vi "CANsub_Phy_Body.vi"(8 "error in (no error)":errorcluster, 11 "Bit_Timing":T1={"brp"=2, "seg1"=63, "seg2"=16, "sjw"=16, "data brp"=2, "data seg1"=15, "data seg2"=4, "data sjw"=4}) -> (0 "error out":errorcluster, 3 "body":string)   [LabVIEW 2021, in "CANsub_Common.lvlib"]
doc: "Builds the CANsub PUT /phy JSON body from the bit timing: listen-only off, auto reset on, error frames on, TX acknowledgements on, nominal and data timing."
uses:
  CANsub_Common.lvlib
  Typedefs/Bit_Timing.ctl
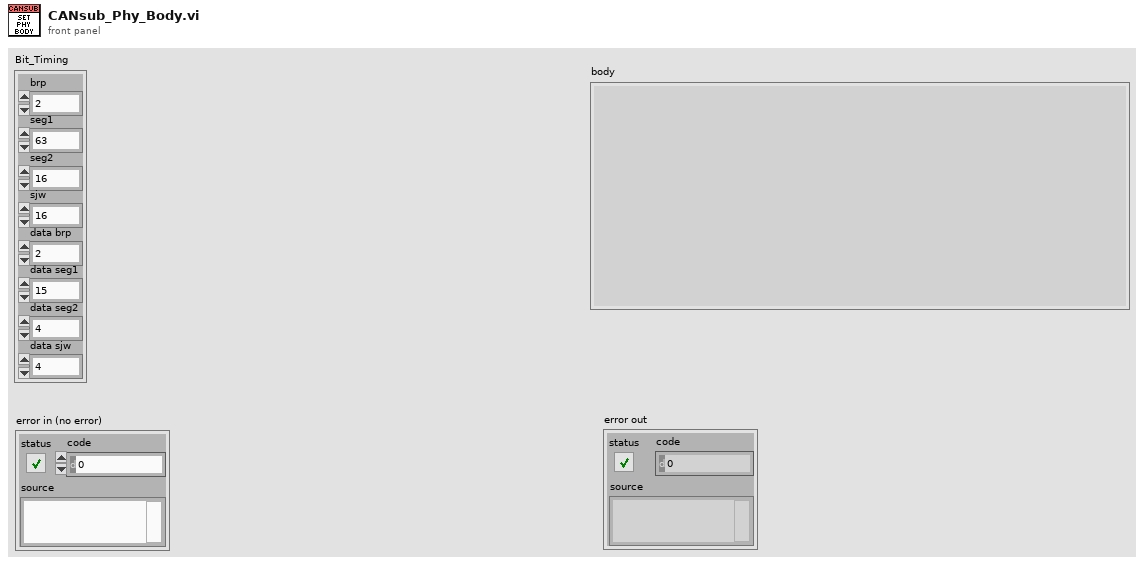
[diagram p1: front panel]
types:
  T1 = typedef "CANsub_Common.lvlib/Bit_Timing.ctl" = cluster{"brp":u16, "seg1":u16, "seg2":u16, "sjw":u16, "data brp":u16, "data seg1":u16, "data seg2":u16, "data sjw":u16}
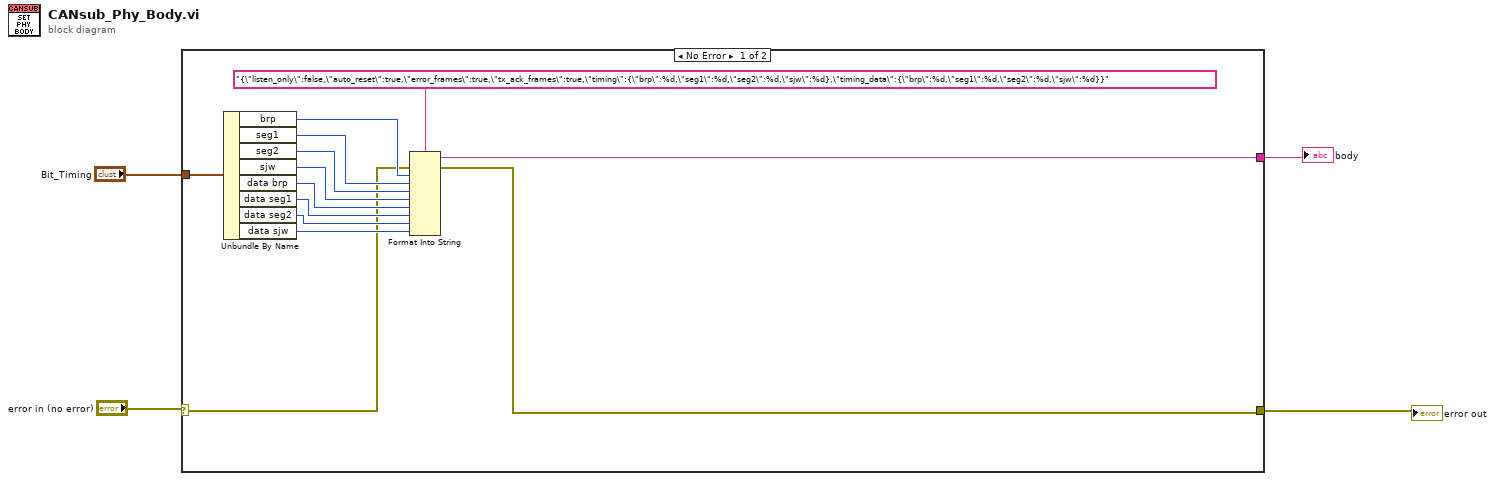
[diagram p0: block diagram]
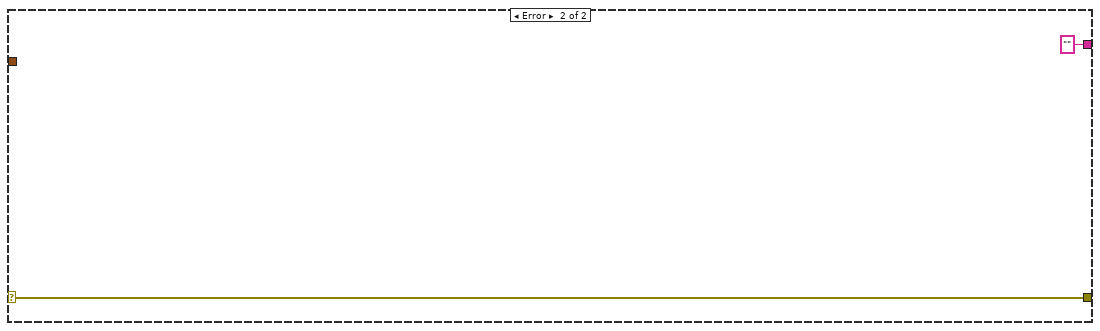
[diagram p2: hidden frame]
diagram:
  n1 = case shown="No Error" "error in (no error)" {
    selector: "error in (no error)" -> [w6 w19]
    tunnel: [w5 w19] -> w4
    tunnel: "Bit_Timing" -> [w17 _]
    tunnel: [w7 ""] -> w1
    frame No Error {
      n2 = Unbundle By Name(w17) -> ("brp"=w15:u16, "seg1"=w14:u16, "seg2"=w13:u16, "sjw"=w12:u16, "data brp"=w11:u16, "data seg1"=w10:u16, "data seg2"=w9:u16, "data sjw"=w8:u16)
      n3 = Format Into String(format string="{\"listen_only\":false,\"auto_reset\":true,\"error_frames\":true,\"tx_ack_frames\":true,\"timing\":{\"brp\":%d,\"seg1\":%d,\"seg2\":%d,\"sjw\":%d},\"timing_data\":{\"brp\":%d,\"seg1\":%d,\"seg2\":%d,\"sjw\":%d}}", error in=w6, w15, w14, w13, w12, w11, w10, w9, w8) -> (resulting string=w7:string, error out=w5:errorcluster)  [unwired: 1 in]
    }
    frame Error {
    }
  }
  "error out" <- w4
  "body" <- w1
